vi "To CSV File.vi"(8 "error in (no error)":errorcluster, 9 "Path":path, 10 "engine configuration":refnum<class "engine configuration.lvclass">, 11 "DAQmx Module Editor Node in":refnum<class "DAQmx Module editor node.lvclass">) -> (0 "error out":errorcluster, 3 "DAQmx Module Editor Node out":refnum<class "DAQmx Module editor node.lvclass">)   [LabVIEW 2015, in "DAQmx Module editor node.lvclass"]
uses:
  DAQmx Module editor node.lvclass
  <vilib>/NI/Module Execution Interface/Engine Configuration/engine configuration.lvclass
  module/configuration/Daqmx Module configuration.lvclass
  <vilib>/NI/Configuration Framework/serializable configuration/NISE_CEF_serializable configuration.lvclass/NISE_CEF_serializable configuration.ctl
  module/configuration/Daqmx Module configuration.lvclass/Daqmx Module configuration.ctl
  <vilib>/NI/Tag Bus/tag/tag descriptor.lvclass/tag descriptor.ctl
  <vilib>/Utility/LVClass/Get LV Class Name.vi
  <vilib>/NI/Configuration Framework/error generator/NISE_error generator.vi
  <vilib>/NI/Tag Bus Module Framework/channel/TBM channel.lvclass
  <vilib>/NI/Configuration Framework/serializable configuration/NISE_CEF_serializable configuration.lvclass
  <vilib>/NI/Tag Bus/tag/tag descriptor.lvclass
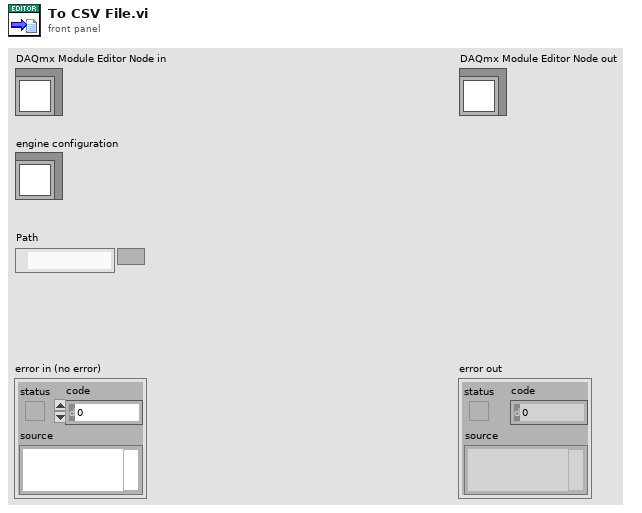
[diagram p1: front panel]
types:
  T1 = typedef "DAQmx Module Configuration.lvclass/Line.ctl" = cluster{"Channel Array":refnum<class "TBM channel.lvclass">[], "Physical Channel":string, "Measurement Type":T2, "Parameters":T3}
  T2 = typedef "DAQmx Module Configuration.lvclass/Measurement Type.ctl" = enum16{"Digital Input", "Digital Output", "Voltage Input", "Voltage Output", "Current Input", "Current Output", "RTD", "Thermocouple", "Strain", "PWM"}
  T3 = typedef "DAQmx Module Configuration.lvclass/Parameters.ctl" = cluster{"Digital Config":cluster{"Invert Lines?":bool}, "Voltage Config":cluster{"Maximum Value (V)":dbl, "Minimum Value (V)":dbl, "in terminal configuration (V)":i32, "out terminal configuration (V)":i32}, "Current Config":cluster{"Maximum Value (A)":dbl, "Minimum Value (A)":dbl, "shunt resistor location":i32, "input terminal configuration (C)":i32, "external shunt resistor value":dbl}, "RTD Config":cluster{"Maximum Value (°C)":dbl, "Minimum Value (°C)":dbl, "resistance configuration":i32, "r0":dbl, "current excitation value":dbl, "rtd type":i32, "current excitation source":i32}, "Thermocouple Config":cluster{"Minimum Value (C)":dbl, "Maximum Value (C)":dbl, "thermocouple type":i32, "cjc source":i32, "cjc value":dbl}, "Strain Config":cluster{"Maximum Value":dbl, "Minimum Value":dbl, "bridge information":cluster{"strain configuration":i32, "lead wire resistance":dbl, "initial bridge voltage":dbl, "voltage excitation source":i32, "voltage excitation value":dbl}, "strain gage information":cluster{"gage factor":dbl, "nominal gage resistance":dbl, "poisson ratio":dbl}}, "PWM Config":cluster{"Idle State":bool}}
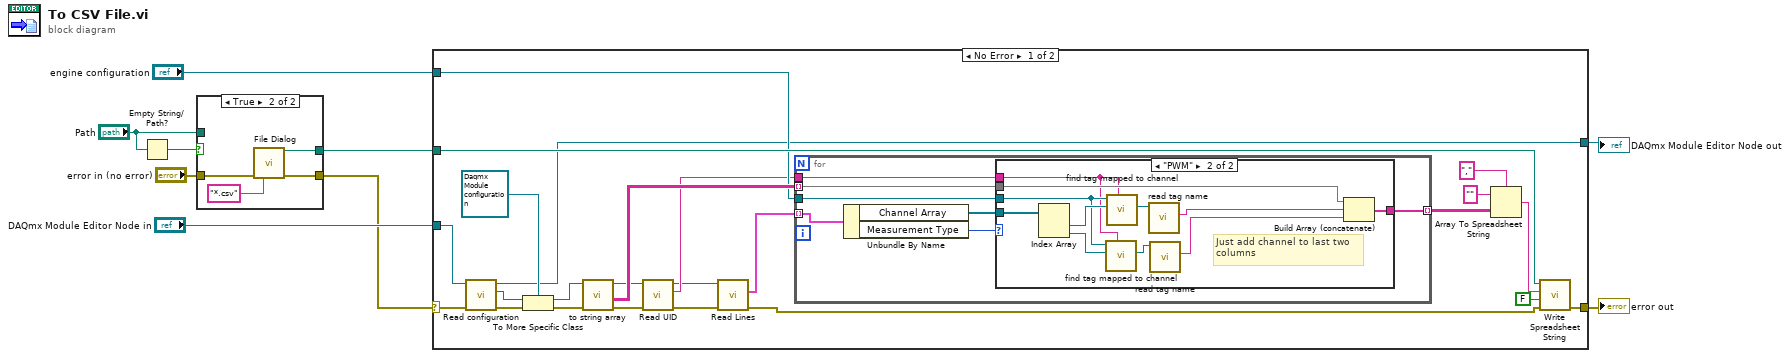
[diagram p0: block diagram]
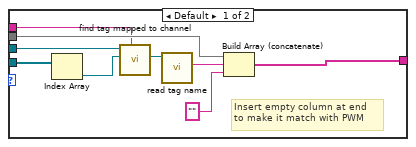
[diagram p3: hidden frame]
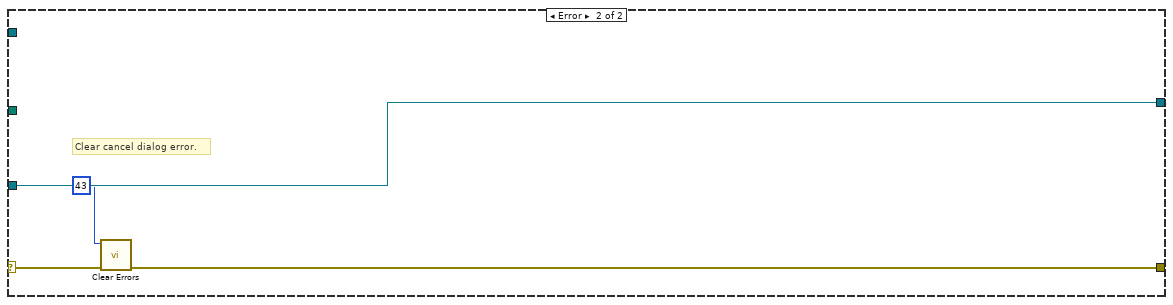
[diagram p4: hidden frame]
diagram:
  n1 = Empty String/Path?(string/path="Path") -> (empty?=w1:bool)
  n2 = case shown="True" w1 {
    tunnel: "error in (no error)" -> [w10 w14]
    tunnel: [w10 w13] -> w4
    tunnel: [w11 w12] -> w3
    tunnel: "Path" -> [w11 _]
    frame False {
    }
    frame True {
      n3 = call "File Dialog"("error in"=w14, "pattern (all files)"="*.csv") -> ("selected path"=w12:path, "error out"=w13:errorcluster)  [unwired: 10 in, 2 out]
    }
  }
  n4 = case shown="No Error" w4 {
    selector: w4 -> [w25 w69]
    tunnel: [w37 w68] -> w9
    tunnel: [w24 w70] -> w6
    tunnel: "DAQmx Module Editor Node in" -> [w26 w70]
    tunnel: w3 -> [w33 _]
    tunnel: "engine configuration" -> [w29 _]
    frame No Error {
      n5 = call-dynamic "Read configuration.vi"("error in"=w25, "Daqmx Module editor node in"=w26) -> ("error out"=w23:errorcluster, "configuration"=w22:refnum<class "NISE_CEF_serializable configuration.lvclass">, "Daqmx Module editor node out"=w24:refnum<class "DAQmx Module editor node.lvclass">)  [unwired: 7 in]
      n6 = To More Specific Class(target class=refnum<class "Daqmx Module configuration.lvclass"> refnum ("Daqmx Module configuration out"), reference=w22, error in=w23) -> (specific class reference=w39:refnum<class "Daqmx Module configuration.lvclass">, error out=w38:errorcluster)
      n7 = call-dynamic "to string array.vi"("error in (no error)"=w38, "module configuration in"=w39) -> ("error out"=w18:errorcluster, "Array"=w31:string[][], "module configuration out"=w19:refnum<class "Daqmx Module configuration.lvclass">)  [unwired: 6 in, 1 out]
      n8 = call <vilib>:"Read UID.vi"("error in"=w18, "configuration in"=w19) -> ("error out"=w17:errorcluster, "instance id"=w28:string, "configuration out"=w21:refnum<class "Daqmx Module configuration.lvclass">)  [unwired: 7 in]
      n9 = call "Read Lines.vi"("error in (no error)"=w17, "Daqmx Module configuration in"=w21) -> ("error out"=w16:errorcluster, "Lines"=w20:T1[])  [unwired: 7 in, 1 out]
      n10 = for {
        tunnel: w31 -> [w44] mode=indexing
        tunnel: [w43] -> w30 mode=indexing
        tunnel: w20 -> [w46] mode=indexing
        tunnel: w29 -> [w45]
        tunnel: w28 -> [w42]
        n11 = Unbundle By Name(w46) -> ("Channel Array"=w41:refnum<class "TBM channel.lvclass">[], "Measurement Type"=w40:T2)
        n12 = case shown="\"PWM\"" w40 {
          tunnel: w45 -> [w55 w60]
          tunnel: w44 -> [w53 w65]
          tunnel: [w51 w64] -> w43
          tunnel: w42 -> [w50 w58]
          tunnel: w41 -> [w49 w63]
          frame Default {
            # "Insert empty column at end\nto make it match with PWM"
            n13 = Index Array(array=w49) -> (element=w48:refnum<class "TBM channel.lvclass">)  [unwired: 1 in]
            n14 = call <vilib>:"find tag mapped to channel.vi"("owner"=w50, "channel"=w48, "engine configuration in"=w55) -> ("tag"=w54:refnum<class "tag descriptor.lvclass">)  [unwired: 6 in, 2 out]
            n15 = call <vilib>:"read tag name.vi"("system tag in"=w54) -> ("name"=w52:string)  [unwired: 8 in, 2 out]
            n16 = Build Array (concatenate)(w53, w52, "" ("element")) -> (w51:string[])
          }
          frame "PWM" {
            # "Just add channel to last two\ncolumns"
            n17 = Index Array(array=w63) -> (element #1=w62:refnum<class "TBM channel.lvclass">, element #2=w61:refnum<class "TBM channel.lvclass">)  [unwired: 2 in]
            n18 = call <vilib>:"find tag mapped to channel.vi"("owner"=w58, "channel"=w61, "engine configuration in"=w60) -> ("tag"=w59:refnum<class "tag descriptor.lvclass">)  [unwired: 6 in, 2 out]
            n19 = call <vilib>:"find tag mapped to channel.vi"("owner"=w58, "channel"=w62, "engine configuration in"=w60) -> ("tag"=w66:refnum<class "tag descriptor.lvclass">)  [unwired: 6 in, 2 out]
            n20 = call <vilib>:"read tag name.vi"("system tag in"=w66) -> ("name"=w57:string)  [unwired: 8 in, 2 out]
            n21 = call <vilib>:"read tag name.vi"("system tag in"=w59) -> ("name"=w56:string)  [unwired: 8 in, 2 out]
            n22 = Build Array (concatenate)(w65, w57, w56) -> (w64:string[])
          }
        }
      }
      n23 = Array To Spreadsheet String(delimiter (Tab)=",", array=w30, 3:"" ("format string")) -> (spreadsheet string=w36:string)
      n24 = call <vilib>:"Write Spreadsheet String.vi"("error in"=w16, "append to file? (new file:F)"=FALSE, "spreadsheet string"=w36, "file path (dialog if empty)"=w33) -> ("error out"=w37:errorcluster)  [unwired: 6 in, 1 out]
    }
    frame Error {
      # "Clear cancel dialog error."
      n25 = call <vilib>:"Clear Errors.vi"("error in (no error)"=w69, "specific error code to clear (0: all)"=43) -> ("error out"=w68:errorcluster)  [unwired: 4 in, 1 out]
    }
  }
  "error out" <- w9
  "DAQmx Module Editor Node out" <- w6
